vi "Own20261012_GetForStop.vi"() -> ()   [LabVIEW 2024]
doc: "本范例演示与For循环相关的常见VI脚本任务。"
panel:
  out "error out":errorcluster caption="错误输出"
  out "stop_id":u32
  in  "for_id":u32
  # "概述：演示ForLoop属性和方法，与VI脚本配合使用，定位和修改For循环。\n操作步骤：\n打开程序框图查看For循环和VI脚本的属性和方法。\n\n注：查看该范例的程序框图，了解VI脚本的概念。本范例不是一个可运行的范例。"
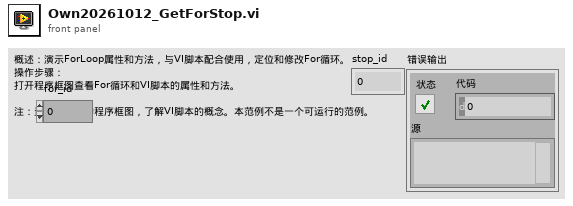
[diagram p1: front panel]
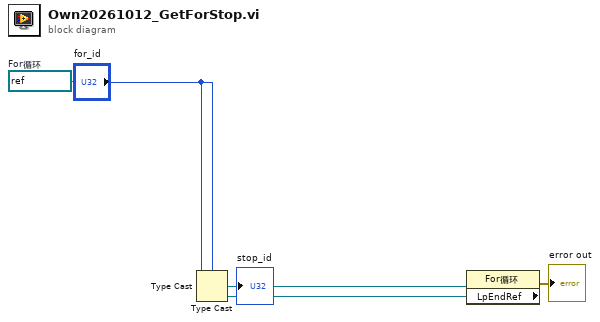
[diagram p0: block diagram]
diagram:
  w5 = refnum<vi> refnum  # For循环
  n1 = Type Cast(type=w5, x="for_id") -> (*(type *) &x=w4:refnum<vi>)
  n2 = property class="For循环"(reference=w4) -> (error out=→"error out":errorcluster, "LpEndRef"=w3:refnum<vi>)  [unwired: 1 in, 1 out]
  n3 = Type Cast(type="for_id", x=w3) -> (*(type *) &x=→"stop_id":u32)
